vi "get status.vi"(8 "error in (no error)":errorcluster, 11 "channel handle":u16 format="%x") -> (0 "error out":errorcluster, 2 "flag names":string[](array[string]), 3 "status":u32 format="%x")   [LabVIEW 2024, in "atsj peakcan basic.lvlib"]
doc: "Gets the current status of a PCAN bus (channel).\n\nCopyright (c) 2025 ATSJ (www.atsj.eu)"
uses:
  atsj peakcan basic.lvlib
  support/x64/PCANBasic.dll
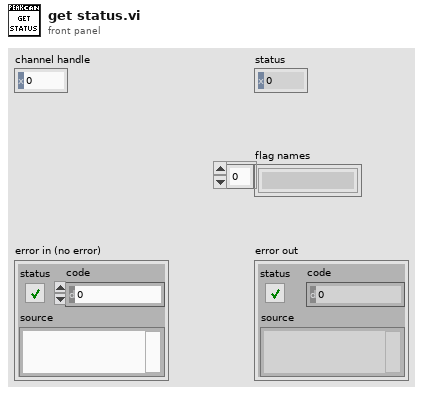
[diagram p1: front panel]
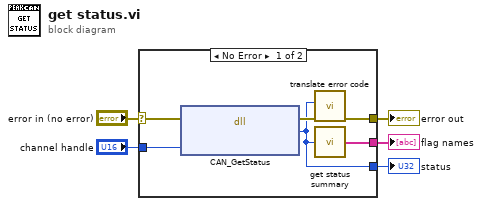
[diagram p0: block diagram]
diagram:
  n1 = case shown="No Error" "error in (no error)" {
    selector: "error in (no error)" -> [w10 w12]
    tunnel: [w8 w12] -> w4
    tunnel: "channel handle" -> [w11 _]
    tunnel: [w7 _] -> w2
    tunnel: [w6 _] -> w1
    frame No Error {
      n2 = dll-call lib="C:/atsj/plateau/atsj-peakcan-basic-for-labview/src/support/x64/PCANBasic.dll" fn="CAN_GetStatus"(error in=w10, "Channel"=w11) -> (error out=w9:errorcluster, "Status"=w7:u32)  [unwired: 3 in, 1 out]
      n3 = call "translate error code.vi"("error in (no error)"=w9, "error code"=w7) -> ("error out"=w8:errorcluster)  [unwired: 9 in]
      n4 = call "get status summary.vi"("status code"=w7) -> ("flag names"=w6:string[])
    }
    frame Error {
    }
  }
  "error out" <- w4
  "status" <- w2
  "flag names" <- w1
